vi "ChopperSignalGenerationForTEST.vi"() -> ()   [LabVIEW 2014]
uses:
  <vilib>/DAQmx/configure/timing.llb/DAQmx Timing (Sample Clock).vi
  <vilib>/DAQmx/write.llb/DAQmx Write (Digital Wfm 1Chan NSamp).vi
  <vilib>/Analysis/NI_AALBase.lvlib
  <vilib>/Analysis/1siggen.llb/Ramp Pattern by Samples.vi
  <vilib>/DAQmx/write.llb/DAQmx Write (Analog 1D Wfm NChan NSamp).vi
  <resource>/objmgr/daqmx.rc
  <vilib>/DAQmx/create/channels.llb/DAQmx Create Channel (CO-Pulse Generation-Frequency).vi
  <vilib>/DAQmx/configure/timing.llb/DAQmx Timing (Implicit).vi
  <vilib>/Waveform/DWDTOps.llb/DWDT Boolean Array to Digital.vi
  <vilib>/DAQmx/create/channels.llb/DAQmx Create Channel (AO-Voltage-Basic).vi
  <vilib>/DAQmx/create/channels.llb/DAQmx Create Channel (DO-Digital Output).vi
panel:
  in  "Source_GATE_DutyCicle (%)":dbl(slide)=3.0 min=0.1 max=99.9 step=0.1 scale=0.0..100.0
  in  "Source_GATE_period (ms)":dbl(slide)=60.0 scale=0.0..1000.0
  out "Faraday IN 2":bool
  in  "Faraday IN":bool
  in  "Chopper ON":bool
  out "Chopper ON 2":bool
  in  "Vmon_L (us)":i32(slide)=920 scale=0.0..3000.0
  in  "Vmon_H (us)":i32(slide)=20 scale=0.0..1000.0
  in  "Vmon_R (us)":i32(slide)=7 scale=0.0..40.0
  in  "Vmon_min (V)":dbl=-8.0 format="%#_13g"
  in  "Vmon_max (V)":dbl format="%#_13g"
  in  "Vmon_F (us)":i32(slide)=8 scale=0.0..40.0
  in  "ACCT_F (us)":i32(slide)=10 scale=0.0..40.0
  in  "ACCT_max (V)":dbl=7.0 format="%#_13g"
  in  "ACCT_min (V)":dbl format="%#_13g"
  in  "ACCT_R (us)":i32(slide)=9 scale=0.0..40.0
  in  "ACCT_H (us)":i32(slide)=20 scale=0.0..1000.0
  in  "ACCT_L (us)":i32(slide)=920 scale=0.0..3000.0
  in  "CH_GATE_H (us)":i32(slide)=34 scale=0.0..100.0
  in  "CH_GATE_L (us)":i32(slide)=920 scale=0.0..3000.0
  in  "Stop Button":bool
  # "Chopper GATE (pins 65,82)"
  # "Vmon (pins 15,16)"
  # "Source GATE (pins 89,82)"
  # "ACCT (pins 31,32)"
  # "Faraday IN (pins 67,82)"
  # "Chopper ON (pins 68,82)"
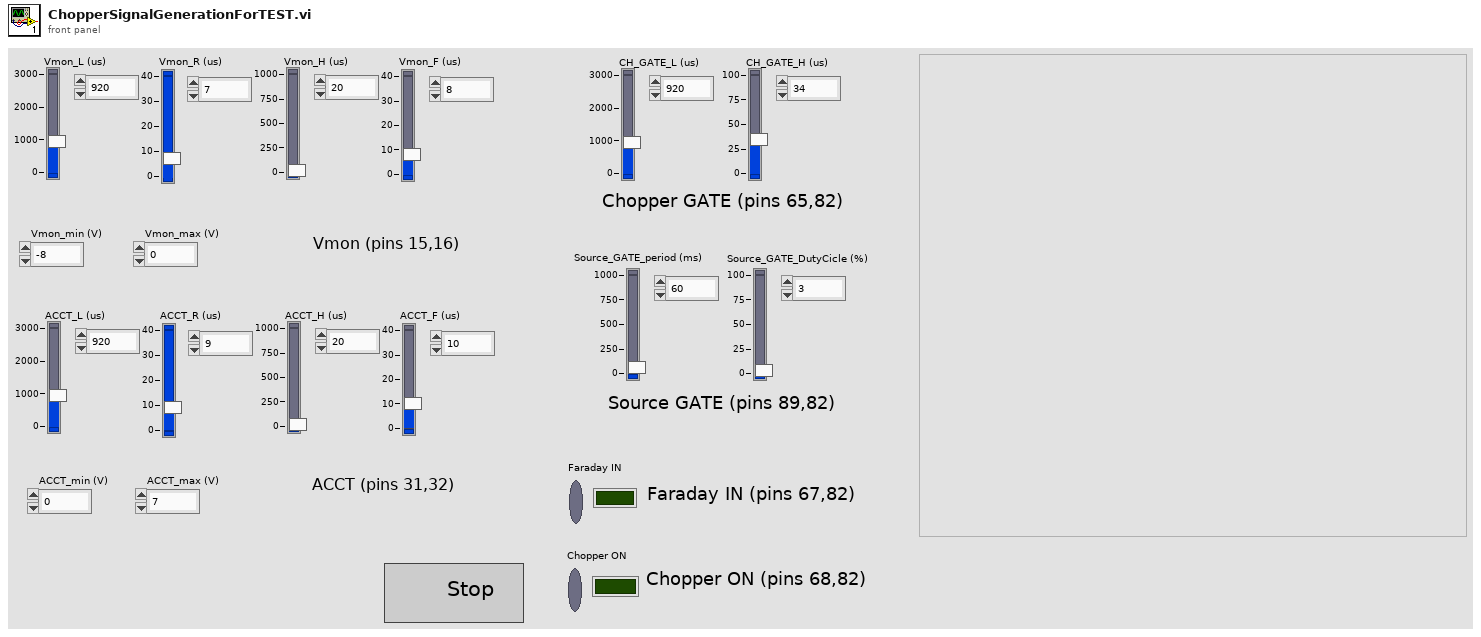
[diagram p1: front panel]
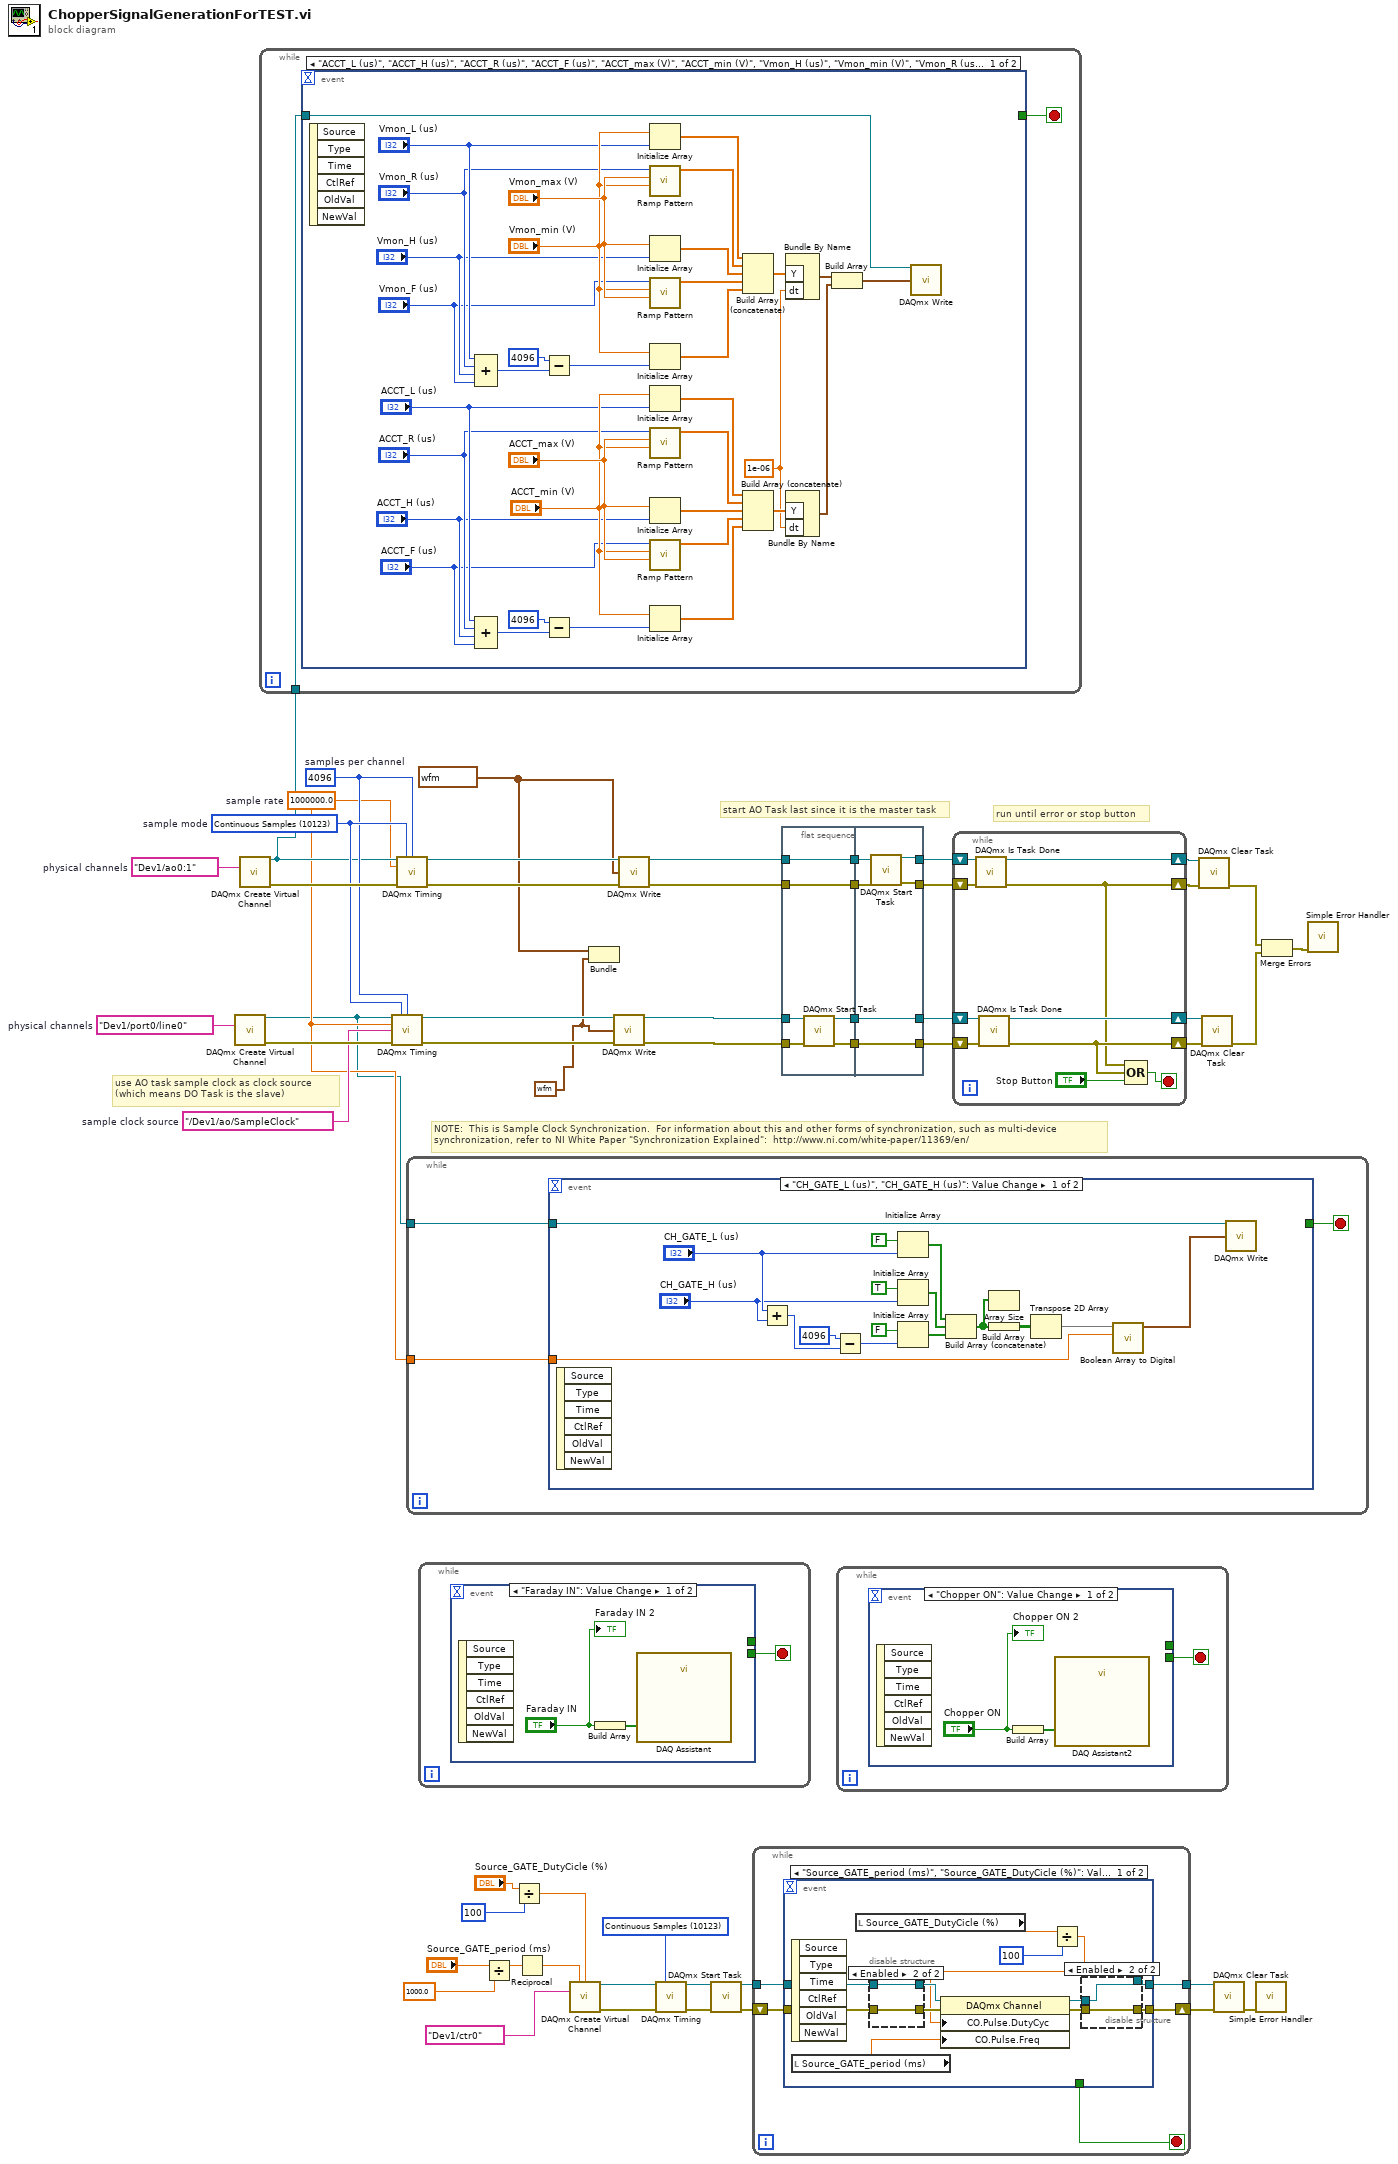
[diagram p0: block diagram]
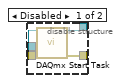
[diagram p2: hidden frame]
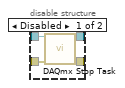
[diagram p3: hidden frame]
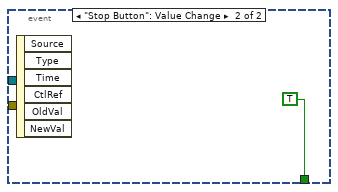
[diagram p4: hidden frame]
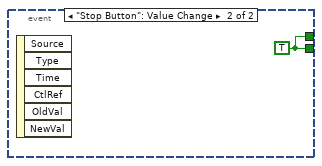
[diagram p5: hidden frame]
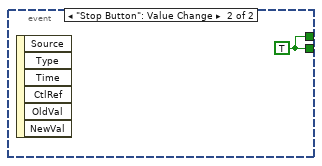
[diagram p6: hidden frame]
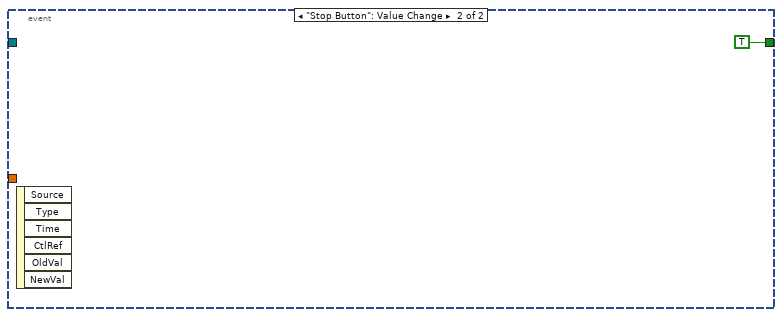
[diagram p7: hidden frame]
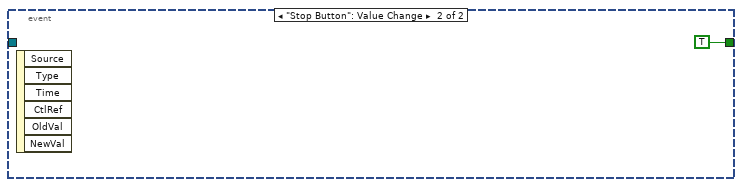
[diagram p8: hidden frame]
diagram:
  w17 = 10123 items=["Finite Samples"=10178, "Continuous Samples"=10123, "Hardware Timed Single Point"=12522] ("sample mode")
  w21 = digitalwaveform {"t0"=timestamp(0 s since 1904-01-01), "dt"=1e-06, "Y"={"transitions"=[], "data"=array4096x1[4096 elements]}} ("digital waveform 2")
  w22 = waveform(dbl)[] [{"t0"=timestamp(0 s since 1904-01-01), "dt"=1e-06, "Y"=array[4096 elements]}, {"t0"=timestamp(0 s since 1904-01-01), "dt"=1e-06, "Y"=array[4096 elements]}] ("appended array 2")
  w38 = tag "/Dev1/ao/SampleClock"  # sample clock source
  w49 = tag "Dev1/port0/line0"  # physical channels
  w39 = 4096  # samples per channel
  w40 = 10123 items=["Finite Samples"=10178, "Continuous Samples"=10123, "Hardware Timed Single Point"=12522]  # sample mode
  w20 = 1000000.0  # sample rate
  w50 = tag "Dev1/ao0:1"  # physical channels
  # "start AO Task last since it is the master task"
  # "NOTE:  This is Sample Clock Synchronization.  For information about this and other forms of synchronization, such as multi-device\nsynchronization, refer to NI White Paper \"Synchronization Explained\":  http://www.ni.com/white-paper/11369/en/"
  # "run until error or stop button"
  # "use AO task sample clock as clock source (which means DO Task is the slave)"
  n1 = call-poly <vilib>:"DAQmx Create Virtual Channel.vi"("lines"=w49) -> ("task out"=w1:refnum<k21>, "error out"=w41:errorcluster)  [unwired: 13 in]
  n2 = call-poly <vilib>:"DAQmx Create Virtual Channel.vi"("physical channels"=w50) -> ("task out"=w26:refnum<k21>, "error out"=w53:errorcluster)  [unwired: 13 in]
  n3 = while {
    tunnel: w26 -> [w55]
    stop <- w54 stop-if-true
    n4 = event shown="[0] \"ACCT_L (us)\", \"ACCT_H (us)\", \"ACCT_R (us)\", \"ACCT_F (us)\", \"ACCT_max (V)\", \"ACCT_min (V)\", \"Vmon_H (us)\", \"Vmon_min (V)\", \"Vmon_R (us)\", \"Vmon_max (V)\", \"Vmon_F (us)\", \"Vmon_L (us)\": Value Change" {
      selector: _ -> [_ _]
      dyn-events: _ -> [_ _]
      timeout: _ -> [_ _]
      tunnel: w55 -> [w81 _]
      tunnel: [_ TRUE ("Stop Button 2")] -> w54
      event "ACCT_L (us)", "ACCT_H (us)", "ACCT_R (us)", "ACCT_F (us)", "ACCT_max (V)", "ACCT_min (V)", "Vmon_H (us)", "Vmon_min (V)", "Vmon_R (us)", "Vmon_max (V)", "Vmon_F (us)", "Vmon_L (us)": Value Change {
        w59 = 1e-06 ("dt")
        n5 = event-data() -> ()  [unwired: 1 in, 6 out]
        n6 = Compound Arithmetic op=ADD("Vmon_L (us)", "Vmon_R (us)", "Vmon_H (us)", "Vmon_F (us)") -> (w61:i32)
        n7 = Compound Arithmetic op=ADD("ACCT_L (us)", "ACCT_R (us)", "ACCT_H (us)", "ACCT_F (us)") -> (w76:i32)
        n8 = Subtract(x=4096, y=w61) -> (x-y=w67:i32)
        n9 = Subtract(x=4096, y=w76) -> (x-y=w83:i32)
        n10 = Initialize Array("Vmon_min (V)", "Vmon_L (us)") -> (w74:dbl[])
        n11 = call-poly <vilib>:"Ramp Pattern.vi"("start"="Vmon_min (V)", "end"="Vmon_max (V)", "samples"="Vmon_R (us)") -> ("Ramp Pattern"=w73:dbl[])  [unwired: 7 in, 1 out]
        n12 = Initialize Array("Vmon_max (V)", "Vmon_H (us)") -> (w72:dbl[])
        n13 = call-poly <vilib>:"Ramp Pattern.vi"("start"="Vmon_max (V)", "end"="Vmon_min (V)", "samples"="Vmon_F (us)") -> ("Ramp Pattern"=w71:dbl[])  [unwired: 7 in, 1 out]
        n14 = Initialize Array("Vmon_min (V)", w67) -> (w68:dbl[])
        n15 = Initialize Array("ACCT_min (V)", "ACCT_L (us)") -> (w90:dbl[])
        n16 = call-poly <vilib>:"Ramp Pattern.vi"("start"="ACCT_min (V)", "end"="ACCT_max (V)", "samples"="ACCT_R (us)") -> ("Ramp Pattern"=w89:dbl[])  [unwired: 7 in, 1 out]
        n17 = Initialize Array("ACCT_max (V)", "ACCT_H (us)") -> (w88:dbl[])
        n18 = call-poly <vilib>:"Ramp Pattern.vi"("start"="ACCT_max (V)", "end"="ACCT_min (V)", "samples"="ACCT_F (us)") -> ("Ramp Pattern"=w87:dbl[])  [unwired: 7 in, 1 out]
        n19 = Initialize Array("ACCT_min (V)", w83) -> (w84:dbl[])
        n20 = Build Array (concatenate)(w74, w73, w72, w71, w68) -> (w60:dbl[])
        n21 = Build Array (concatenate)(w90, w89, w88, w87, w84) -> (w75:dbl[])
        n22 = Bundle By Name("Y"=w60, "dt"=w59) -> (w58:waveform(dbl))  [unwired: 1 in]
        n23 = Bundle By Name("Y"=w75, "dt"=w59) -> (w57:waveform(dbl))  [unwired: 1 in]
        n24 = Build Array(w58, w57) -> (w56:waveform(dbl)[])
        n25 = call-poly <vilib>:"DAQmx Write.vi"("task/channels in"=w81, "data"=w56) -> ()  [unwired: 11 in, 3 out]
      }
      event "Stop Button": Value Change {
        n26 = event-data() -> ()  [unwired: 1 in, 6 out]
      }
    }
  }
  n27 = call-poly <vilib>:"DAQmx Timing.vi"("task/channels in"=w1, "sample mode"=w40, "samples per channel"=w39, "rate"=w20, "source"=w38, "error in"=w41) -> ("task out"=w25:refnum<k21>, "error out"=w42:errorcluster)  [unwired: 8 in]
  n28 = call-poly <vilib>:"DAQmx Timing.vi"("task/channels in"=w26, "sample mode"=w40, "samples per channel"=w39, "rate"=w20, "error in"=w53) -> ("task out"=w37:refnum<k21>, "error out"=w36:errorcluster)  [unwired: 9 in]
  n29 = while {
    tunnel: w20 -> [w94]
    tunnel: w1 -> [w93]
    stop <- w92 stop-if-true
    n30 = event shown="[0] \"CH_GATE_L (us)\", \"CH_GATE_H (us)\": Value Change" {
      selector: _ -> [_ _]
      dyn-events: _ -> [_ _]
      timeout: _ -> [_ _]
      tunnel: w94 -> [w105 _]
      tunnel: w93 -> [w96 _]
      tunnel: [_ TRUE ("Stop Button 3")] -> w92
      event "CH_GATE_L (us)", "CH_GATE_H (us)": Value Change {
        n31 = event-data() -> ()  [unwired: 1 in, 6 out]
        n32 = Add(x="CH_GATE_L (us)", y="CH_GATE_H (us)") -> (x+y=w99:i32)
        n33 = Subtract(x=4096, y=w99) -> (x-y=w97:i32)
        n34 = Initialize Array(FALSE, "CH_GATE_L (us)") -> (w109:bool[])
        n35 = Initialize Array(TRUE, "CH_GATE_H (us)") -> (w108:bool[])
        n36 = Initialize Array(FALSE, w97) -> (w101:bool[])
        n37 = Build Array (concatenate)(w109, w108, w101) -> (w106:bool[])
        n38 = Array Size(array=w106) -> ()  [unwired: 1 out]
        n39 = Build Array(w106) -> (w107:bool[][])
        n40 = Transpose 2D Array(2D array=w107) -> (transposed array=w104:bool[][])
        n41 = call-poly <vilib>:"Boolean Array to Digital.vi"("sample rate"=w105, "boolean array"=w104) -> ("digital waveform"=w95:digitalwaveform)  [unwired: 8 in, 1 out]
        n42 = call-poly <vilib>:"DAQmx Write.vi"("task/channels in"=w96, "data"=w95) -> ()  [unwired: 11 in, 3 out]
      }
      event "Stop Button": Value Change {
        n43 = event-data() -> ()  [unwired: 1 in, 6 out]
      }
    }
  }
  n44 = while {
    stop <- w113 stop-if-true
    n45 = event shown="[0] \"Faraday IN\": Value Change" {
      selector: _ -> [_ _]
      dyn-events: _ -> [_ _]
      timeout: _ -> [_ _]
      tunnel: [_ w116] -> _
      tunnel: [_ w116] -> w113
      event "Faraday IN": Value Change {
        n46 = event-data() -> ()  [unwired: 1 in, 6 out]
        n47 = Build Array("Faraday IN") -> (w114:bool[])
        n48 = call "DAQ Assistant"("data"=w114) -> ()  [unwired: 17 in, 2 out]
        "Faraday IN 2" <- "Faraday IN"
      }
      event "Stop Button": Value Change {
        w116 = TRUE
        n49 = event-data() -> ()  [unwired: 1 in, 6 out]
      }
    }
  }
  n50 = Divide(x="Source_GATE_period (ms)", y=1000.0) -> (x/y=w4:dbl)
  n51 = Divide(x="Source_GATE_DutyCicle (%)", y=100) -> (x/y=w6:dbl)
  n52 = Reciprocal(x=w4) -> (1/x=w2:dbl)
  n53 = call-poly <vilib>:"DAQmx Create Virtual Channel.vi"("frequency"=w2, "duty cycle"=w6, "counter"=tag "Dev1/ctr0" ("Physical Channels")) -> ("task out"=w18:refnum<k21>, "error out"=w19:errorcluster)  [unwired: 6 in, 5 out]
  n54 = Bundle("appended array 2"=w22, "digital waveform 2"=w21) -> ()  [unwired: 1 in, 1 out]
  n55 = call-poly <vilib>:"DAQmx Write.vi"("task/channels in"=w25, "data"=w21, "error in"=w42) -> ("task out"=w43:refnum<k21>, "error out"=w44:errorcluster)  [unwired: 10 in, 1 out]
  n56 = call-poly <vilib>:"DAQmx Write.vi"("task/channels in"=w37, "data"=w22, "error in"=w36) -> ("task out"=w33:refnum<k21>, "error out"=w32:errorcluster)  [unwired: 10 in, 1 out]
  n57 = call-poly <vilib>:"DAQmx Timing.vi"("task/channels in"=w18, "sample mode"=w17, "error in"=w19) -> ("task out"=w15:refnum<k21>, "error out"=w16:errorcluster)  [unwired: 11 in]
  n58 = call <vilib>:"DAQmx Start Task.vi"("task/channels in"=w15, "error in"=w16) -> ("task out"=w10:refnum<k21>, "error out"=w11:errorcluster)  [unwired: 12 out]
  n59 = while {
    tunnel: w10 -> [w121]
    tunnel: [w120] -> w12
    shift-right: [w119] -> w13
    shift-left: w11 -> [w118]
    stop <- w117 stop-if-true
    n60 = event shown="[0] \"Source_GATE_period (ms)\", \"Source_GATE_DutyCicle (%)\": Value Change" {
      selector: _ -> [_ _]
      dyn-events: _ -> [_ _]
      timeout: _ -> [_ _]
      tunnel: w121 -> [w133 _]
      tunnel: [w122 _] -> w120
      tunnel: [w132 _] -> w119
      tunnel: w118 -> [w131 _]
      tunnel: [_ TRUE] -> w117
      event "Source_GATE_period (ms)", "Source_GATE_DutyCicle (%)": Value Change {
        n61 = event-data() -> ()  [unwired: 1 in, 6 out]
        n62 = local read "Source_GATE_period (ms)"() -> (w123:dbl)
        n63 = local read "Source_GATE_DutyCicle (%)"() -> (w126:dbl)
        n64 = disable-structure shown="Enabled" {
          disable-tunnel: w133 -> [w143 w145]
          disable-tunnel: w131 -> [w142 w144]
          disable-tunnel: [w141 w145] -> w130
          disable-tunnel: [w140 w144] -> w128
          frame Disabled {
            n65 = call <vilib>:"DAQmx Stop Task.vi"("task/channels in"=w143, "error in"=w142) -> ("task out"=w141:refnum<k21>, "error out"=w140:errorcluster)  [unwired: 12 out]
          }
          frame Enabled {
          }
        }
        n66 = Divide(x=w126, y=100) -> (x/y=w124:dbl)
        n67 = property class="DAQmx Channel"(reference=w130, error in=w128, "CO.Pulse.DutyCyc"=w124, "CO.Pulse.Freq"=w123) -> (reference out=w129:refnum<k21>, error out=w127:errorcluster)
        n68 = disable-structure shown="Enabled" {
          disable-tunnel: [w136 w138] -> w132
          disable-tunnel: w129 -> [w135 w139]
          disable-tunnel: w127 -> [w134 w138]
          disable-tunnel: [w137 w139] -> w122
          frame Disabled {
            n69 = call <vilib>:"DAQmx Start Task.vi"("task/channels in"=w135, "error in"=w134) -> ("task out"=w137:refnum<k21>, "error out"=w136:errorcluster)  [unwired: 12 out]
          }
          frame Enabled {
          }
        }
      }
      event "Stop Button": Value Change {
        n70 = event-data() -> ()  [unwired: 1 in, 6 out]
      }
    }
  }
  n71 = flat-sequence {
    tunnel: w44 -> [w150]
    tunnel: w43 -> [w149]
    tunnel: [w152] -> w35
    tunnel: [w151] -> w34
    tunnel: w33 -> [w148]
    tunnel: w32 -> [w147]
    tunnel: [w148] -> w24
    tunnel: [w147] -> w23
    tunnel: [w157] -> w45
    tunnel: [w158] -> w46
    tunnel: w35 -> [w158]
    tunnel: w34 -> [w157]
    tunnel: [w154] -> w31
    tunnel: [w153] -> w30
    tunnel: w24 -> [w156]
    tunnel: w23 -> [w155]
    frame #0 {
      n72 = call <vilib>:"DAQmx Start Task.vi"("task/channels in"=w149, "error in"=w150) -> ("task out"=w151:refnum<k21>, "error out"=w152:errorcluster)  [unwired: 12 in]
    }
    frame #1 {
      n73 = call <vilib>:"DAQmx Start Task.vi"("task/channels in"=w156, "error in"=w155) -> ("task out"=w154:refnum<k21>, "error out"=w153:errorcluster)  [unwired: 12 in]
    }
  }
  n74 = while {
    stop <- w159 stop-if-true
    n75 = event shown="[0] \"Chopper ON\": Value Change" {
      selector: _ -> [_ _]
      dyn-events: _ -> [_ _]
      timeout: _ -> [_ _]
      tunnel: [_ w162] -> _
      tunnel: [_ w162] -> w159
      event "Chopper ON": Value Change {
        n76 = event-data() -> ()  [unwired: 1 in, 6 out]
        n77 = Build Array("Chopper ON") -> (w160:bool[])
        n78 = call "DAQ Assistant2"("data"=w160) -> ()  [unwired: 17 in, 2 out]
        "Chopper ON 2" <- "Chopper ON"
      }
      event "Stop Button": Value Change {
        w162 = TRUE
        n79 = event-data() -> ()  [unwired: 1 in, 6 out]
      }
    }
  }
  n80 = while {
    shift-right: [w165] -> w48
    shift-left: w46 -> [w170]
    shift-right: [w171] -> w47
    shift-left: w45 -> [w169]
    shift-right: [w172] -> w52
    shift-left: w31 -> [w168]
    shift-right: [w164] -> w51
    shift-left: w30 -> [w167]
    stop <- w163 stop-if-true
    n81 = call <vilib>:"DAQmx Is Task Done.vi"("task/channels in"=w168, "error in"=w167) -> ("task out"=w172:refnum<k21>, "error out"=w164:errorcluster)  [unwired: 11 in, 1 out]
    n82 = call <vilib>:"DAQmx Is Task Done.vi"("task/channels in"=w169, "error in"=w170) -> ("task out"=w171:refnum<k21>, "error out"=w165:errorcluster)  [unwired: 11 in, 1 out]
    n83 = Compound Arithmetic op=OR(w164, w165, "Stop Button") -> (w163:bool)
  }
  n84 = call <vilib>:"DAQmx Clear Task.vi"("task in"=w52, "error in"=w51) -> ("error out"=w28:errorcluster)  [unwired: 13 in]
  n85 = call <vilib>:"DAQmx Clear Task.vi"("task in"=w47, "error in"=w48) -> ("error out"=w27:errorcluster)  [unwired: 13 in]
  n86 = call <vilib>:"DAQmx Clear Task.vi"("task in"=w12, "error in"=w13) -> ("error out"=w14:errorcluster)  [unwired: 13 out]
  n87 = call <vilib>:"Simple Error Handler.vi"("error in (no error)"=w14) -> ()  [unwired: 4 in, 5 out]
  n88 = Merge Errors(w28, w27) -> (w29:errorcluster)
  n89 = call <vilib>:"Simple Error Handler.vi"("error in (no error)"=w29) -> ()  [unwired: 4 in, 5 out]
